vi "Write Active Path.vi"(8 "error in (no error)":errorcluster, 10 "Path Settings.lvclass":refnum<class "Path Settings.lvclass">, 11 "Setting Database in":refnum<class "Setting Database.lvclass">) -> (0 "error out":errorcluster, 3 "Setting Database out":refnum<class "Setting Database.lvclass">)   [LabVIEW 2019, in "Setting Database.lvclass"]
uses:
  Setting Database.lvclass
  Path Settings/Path Settings.lvclass
  Setting Database.lvclass/Setting Database.ctl
  C:/Users/Albro/Documents/GitHub/AFM-Lithography/lvsrc/Classes/Settings/ObjectSettings/ObjectSettings.lvclass
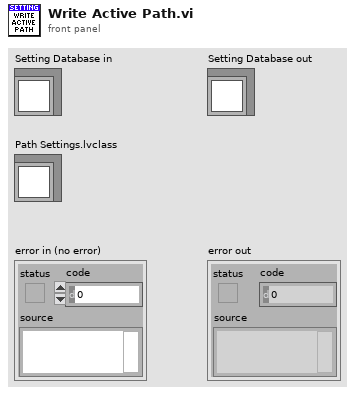
[diagram p1: front panel]
types:
  T1 = cluster{"Path":string, "Funnel":string, "Rectangle":string, "Dot":string}
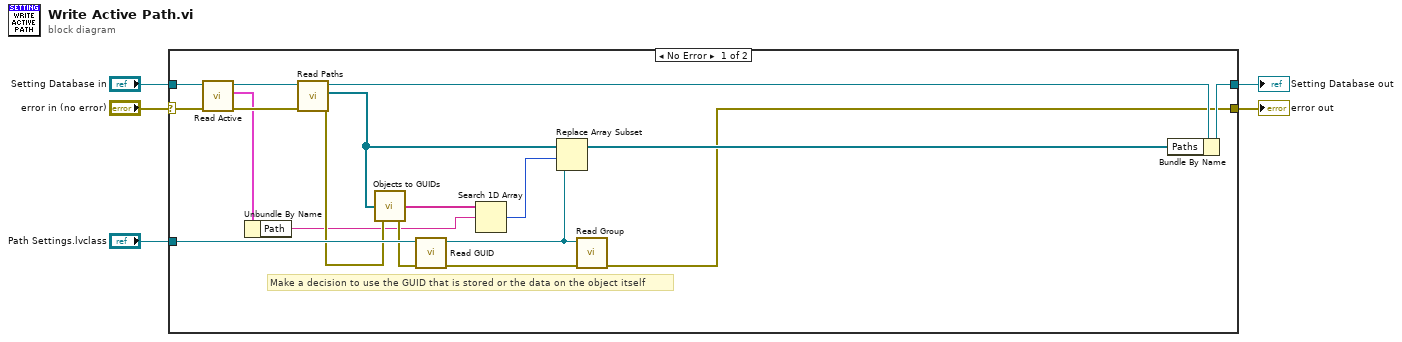
[diagram p0: block diagram]
diagram:
  n1 = case shown="No Error" "error in (no error)" {
    selector: "error in (no error)" -> [w22 w25]
    tunnel: [w15 w25] -> w4
    tunnel: [w21 w24] -> w2
    tunnel: "Setting Database in" -> [w18 w24]
    tunnel: "Path Settings.lvclass" -> [w10 _]
    frame No Error {
      # "Make a decision to use the GUID that is stored or the data on the object itself"
      n2 = call "Read Active.vi"("error in (no error)"=w22, "Setting Database in"=w18) -> ("error out"=w23:errorcluster, "Active"=w17:T1, "Setting Database out"=w19:refnum<class "Setting Database.lvclass">)  [unwired: 7 in]
      n3 = Unbundle By Name(w17) -> ("Path"=w6:string)
      n4 = call "Read Paths.vi"("error in (no error)"=w23, "Setting Database in"=w19) -> ("error out"=w8:errorcluster, "Paths"=w14:refnum<class "Path Settings.lvclass">[], "Setting Database out"=w20:refnum<class "Setting Database.lvclass">)  [unwired: 7 in]
      n5 = call "Objects to GUIDs.vi"("error in (no error)"=w8, "Objects"=w14) -> ("error out"=w7:errorcluster, "GUIDs"=w12:string[])  [unwired: 2 in]
      n6 = call-dynamic "Read GUID.vi"("error in (no error)"=w7, "ObjectSettings in"=w10) -> ("error out"=w13:errorcluster, "ObjectSettings out"=w11:refnum<class "Path Settings.lvclass">)  [unwired: 7 in, 1 out]
      n7 = Search 1D Array(1D array=w12, element=w6) -> (index of element=w9:i32)  [unwired: 1 in]
      n8 = Replace Array Subset(array=w14, new element=w11, index=w9) -> (w16:refnum<class "Path Settings.lvclass">[])
      n9 = call-dynamic "Read Group.vi"("error in (no error)"=w13, "ObjectSettings in"=w11) -> ("error out"=w15:errorcluster)  [unwired: 7 in, 2 out]
      n10 = Bundle By Name(cluster=w20, "Paths"=w16) -> (w21:refnum<class "Setting Database.lvclass">)
    }
    frame Error {
    }
  }
  "error out" <- w4
  "Setting Database out" <- w2
